vi "Get Case Structure (by Name).vi"(8 "error in (no error)":errorcluster, 10 "Case Structure name":string, 11 "VI ref in":refnum<vi>) -> (0 "error out":errorcluster, 1 "Found ?":bool, 2 "CaseStructure out":refnum<vi>, 3 "VI ref out":refnum<vi>)   [LabVIEW 2019, in "gRPC Template Creation Utility.lvlib"]
uses:
  gRPC Template Creation Utility.lvlib
  <vilib>/Utility/traverseref.llb/TRef TravTarget.ctl
  <vilib>/Utility/traverseref.llb/VI Scripting - Traverse.lvlib
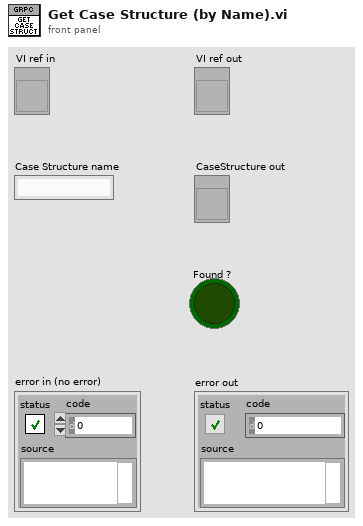
[diagram p1: front panel]
types:
  T1 = typedef "TRef TravTarget.ctl" = enum16{"FP", "BD", "Other"}
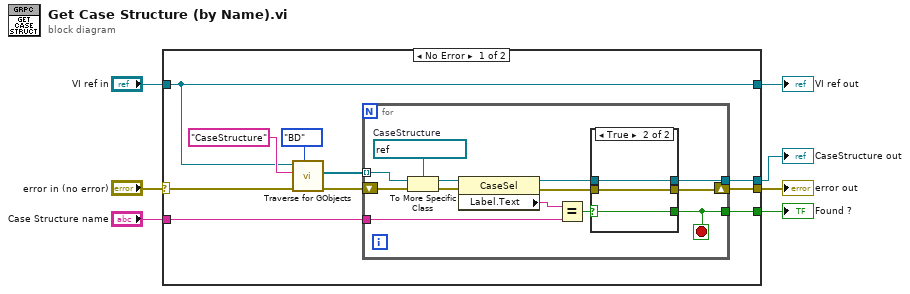
[diagram p0: block diagram]
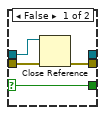
[diagram p2: hidden frame]
diagram:
  n1 = case shown="No Error" "error in (no error)" {
    selector: "error in (no error)" -> [w11 w39]
    tunnel: [w17 _] -> w7
    tunnel: "Case Structure name" -> [w16 _]
    tunnel: "VI ref in" -> [w8 w38]
    tunnel: [w12 _] -> w4
    tunnel: [w9 w39] -> w2
    tunnel: [w8 w38] -> w1
    frame No Error {
      n2 = call <vilib>:"Traverse for GObjects.vi"("Traverse Target"=TRef_TravTarget."BD", "error in (no error)"=w11, "Class Name"="CaseStructure", "VI Refnum"=w8) -> ("error out"=w10:errorcluster, "References"=w15:refnum<vi>[])  [unwired: 4 in, 2 out]
      n3 = for {
        tunnel: w15 -> [w28] mode=indexing
        tunnel: w16 -> [w26]
        tunnel: [w23] -> w17
        tunnel: [w19] -> w12
        shift-right: [w18] -> w9
        shift-left: w10 -> [w22]
        stop <- w19 stop-if-true
        w30 = refnum<vi> refnum  # CaseStructure
        n4 = To More Specific Class(target class=w30, reference=w28, error in=w22) -> (specific class reference=w29:refnum<vi>, error out=w20:errorcluster)
        n5 = property class="CaseSel"(reference=w29, error in=w20) -> (reference out=w24:refnum<vi>, error out=w21:errorcluster, "Label.Text"=w27:string)
        n6 = Equal?(x=w27, y=w26) -> (x = y?=w25:bool)
        n7 = case shown="True" w25 {
          selector: w25 -> [w31 w35]
          tunnel: w24 -> [w34 w37]
          tunnel: [_ w37] -> w23
          tunnel: [w31 w35] -> w19
          tunnel: w21 -> [w33 w36]
          tunnel: [w32 w36] -> w18
          frame False {
            n8 = Close Reference(reference=w34, error in (no error)=w33) -> (error out=w32:errorcluster)
          }
          frame True {
          }
        }
      }
    }
    frame Error {
    }
  }
  "CaseStructure out" <- w7
  "VI ref out" <- w1
  "Found ?" <- w4
  "error out" <- w2
